vi "Initialization.vi"(8 "error in (no error)":errorcluster, 9 "UI Refs":T1, 10 "user event":T2, 11 "4way Leakage in":refnum<class "Leakage.lvclass">) -> (0 "error out":errorcluster, 3 "4way Leakage out":refnum<class "Leakage.lvclass">)   [LabVIEW 2025, in "Flow Grind.lvlib" / "Leakage.lvclass"]
uses:
  Leakage.lvclass
  Users/Public/Documents/Sandia National Labs/TSS Plugin/CEF.lvlibp/Node/UserEventRef.ctl
  Users/Public/Documents/Sandia National Labs/TSS Plugin/Tests/XY Plotter.lvlibp/XY  Plotter/XY Plotter.lvclass
  Users/Public/Documents/Sandia National Labs/TSS Plugin/CEF.lvlibp/Node/CEF_Node.lvclass
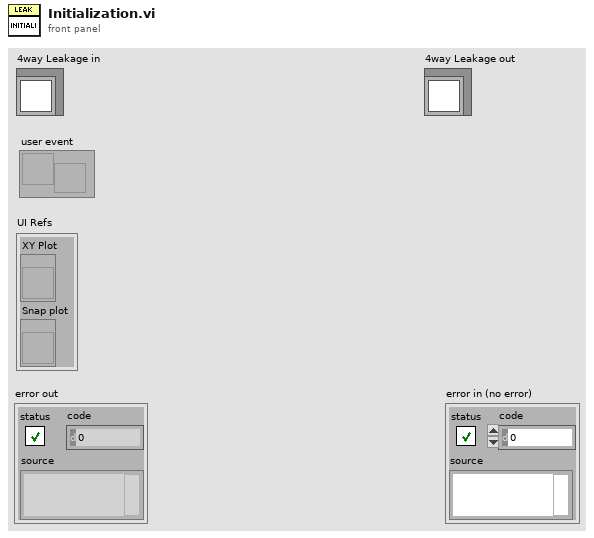
[diagram p1: front panel]
types:
  T1 = cluster{"XY Plot":refnum<vi>, "Snap plot":refnum<vi>}
  T2 = typedef "CEF.lvlibp/CEF_Node.lvclass/UserEventRef.ctl" = refnum<user-event>
  T3 = cluster{"Name":string, "Color":u32, "Style":u8, "Point Style":u8, "Name Visible":bool, "Allow Drag":bool, "Annotation Mode":u32, "Plot":i32, "Index":i32, "Position":cluster{"X":dbl, "Y":dbl}, "X Scale":u32, "Y Scale":u32, "Show Arrow":bool, "Lock Name":bool, "Plot Area":i32, "Label Offset":cluster{"X":dbl, "Y":dbl}}
  T4 = cluster{"Name":string, "Color":u32, "Style":u8, "Point Style":u8, "Name Visible":bool, "Allow Drag":bool, "Annotation Mode":u32, "Plot":i32, "Index":i32, "Position":cluster{"X":dbl, "Y":dbl}, "X Scale":u32, "Y Scale":u32, "Show Arrow":bool, "Lock Name":bool, "Plot Area":i32, "Label Offset":cluster{"X":dbl, "Y":dbl}}[]
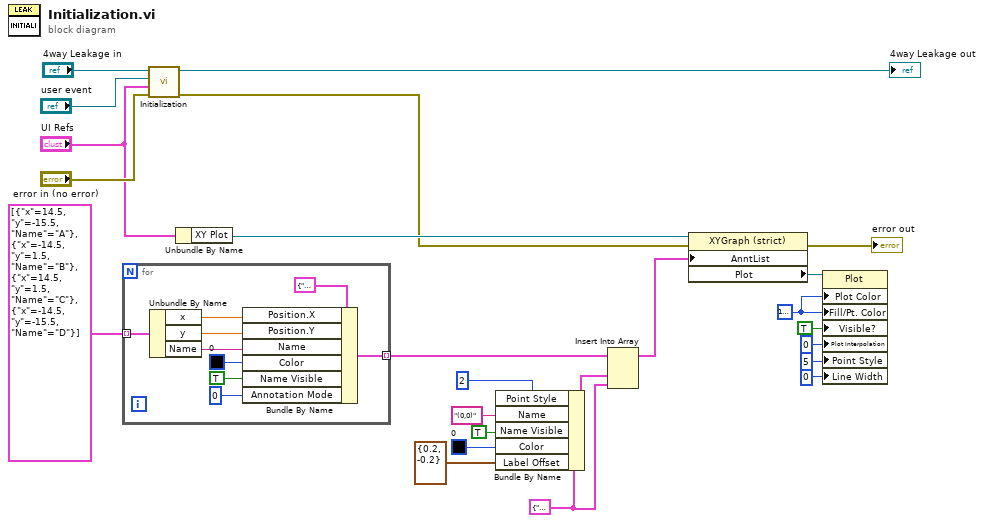
[diagram p0: block diagram]
diagram:
  w2 = T3 {"Name"="", "Color"=0, "Style"=0, "Point Style"=0, "Name Visible"=FALSE, "Allow Drag"=FALSE, "Annotation Mode"=0, "Plot"=0, "Index"=0, "Position"={"X"=0.0, "Y"=0.0}, "X Scale"=0, "Y Scale"=0, "Show Arrow"=FALSE, "Lock Name"=FALSE, "Plot Area"=0, "Label Offset"={"X"=0.0, "Y"=0.0}} ("new element/subarray")
  w16 = u32 16777224 ("Plot Color")
  n1 = for {
    tunnel: cluster{"x":dbl, "y":dbl, "Name":string}[] [{"x"=14.5, "y"=-15.5, "Name"="A"}, {"x"=-14.5, "y"=1.5, "Name"="B"}, {"x"=14.5, "y"=1.5, "Name"="C"}, {"x"=-14.5, "y"=-15.5, "Name"="D"}] -> [w28] mode=indexing
    tunnel: [w29] -> w10 mode=indexing
    n2 = Unbundle By Name(w28) -> ("x"=w26:dbl, "y"=w25:dbl, "Name"=w27:string)
    n3 = Bundle By Name(cluster=T3 {"Name"="", "Color"=0, "Style"=0, "Point Style"=0, "Name Visible"=FALSE, "Allow Drag"=FALSE, "Annotation Mode"=0, "Plot"=0, "Index"=0, "Position"={"X"=0.0, "Y"=0.0}, "X Scale"=0, "Y Scale"=0, "Show Arrow"=FALSE, "Lock Name"=FALSE, "Plot Area"=0, "Label Offset"={"X"=0.0, "Y"=0.0}}, "Position.X"=w26, "Position.Y"=w25, "Name"=w27, "Color"=u32 0, "Name Visible"=TRUE, "Annotation Mode"=u32 0) -> (w29:T3)
  }
  n4 = call-parent "Initialization.vi"("error in"="error in (no error)", "UI Refs"="UI Refs", "user event"="user event", "XY Plotter"="4way Leakage in") -> ("error out"=w12:errorcluster, "XY Plotter out"=→"4way Leakage out":refnum<class "Leakage.lvclass">)  [unwired: 6 in]
  n5 = Unbundle By Name("UI Refs") -> ("XY Plot"=w14:refnum<vi>)
  n6 = Bundle By Name(cluster=w2, "Point Style"=u8 2, "Name"="(0,0)", "Name Visible"=TRUE, "Color"=u32 0, "Label Offset"=cluster{"X":dbl, "Y":dbl} {"X"=0.2, "Y"=-0.2}) -> (w3:T3)
  n7 = Insert Into Array(array=w10, new element #1=w3, new element #2=w2) -> (w9:T4)  [unwired: 1 in]
  n8 = property class="XYGraph (strict)"(reference=w14, error in=w12, "AnntList"=w9) -> (error out=→"error out":errorcluster, "Plot"=w13:refnum<vi>)  [unwired: 1 out]
  n9 = property class="Plot"(reference=w13, "Plot Color"=w16, "Fill/Pt. Color"=w16, "Visible?"=TRUE ("Visible"), "Plot Interpolation"=u8 0, "Point Style"=u8 5, "Line Width"=u8 0) -> ()  [unwired: 1 in, 2 out]
